vi "Finalize.vi"(8 "error in":errorcluster, 11 "Shared Resources in":refnum<class "Shared Resources.lvclass">) -> (0 "error out":errorcluster, 3 "Shared Resources out":refnum<class "Shared Resources.lvclass">)   [LabVIEW 2020, in "AIM ARINC 429 Engine.lvlib" / "Implementation.lvlib" / "Shared Resources.lvclass"]
uses:
  Shared Resources.lvclass
  Shared Resources.lvclass/Shared Resources.ctl
  Hardware API/AIM ARINC 429 Hardware API.lvlib
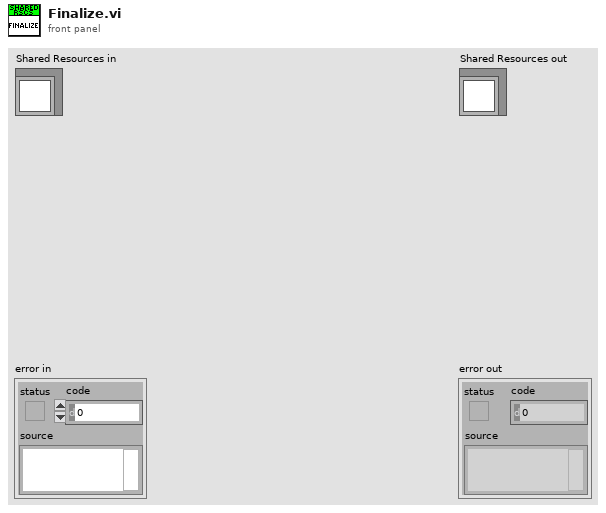
[diagram p1: front panel]
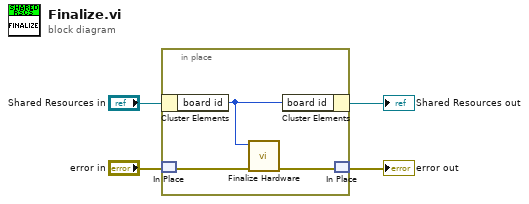
[diagram p0: block diagram]
diagram:
  n1 = in-place {
    n2 = in-place-cluster #1("Shared Resources in") -> ("board id"=w5:u32)
    n3 = in-place-match #2("error in") -> (w7:errorcluster)
    n4 = call "Finalize Hardware.vi"("error in"=w7, "board identifier"=w5) -> ("error out"=w6:errorcluster)  [unwired: 9 in]
    n5 = in-place-cluster #1("board id"=w5) -> (→"Shared Resources out":refnum<class "Shared Resources.lvclass">)
    n6 = in-place-match #2(w6) -> (→"error out":errorcluster)
  }
